vi "GetAncestorClass.vi"(1 "LabVIEWClass":refnum<vi>, 5 "error in (no error)":errorcluster) -> (15 "Ancestor":refnum<vi>, 19 "error out":errorcluster)   [LabVIEW 2017, in "G#IDE.lvlib" / "LibraryLib.lvlib"]
uses:
  LibraryLib.lvlib
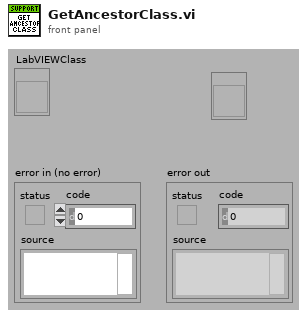
[diagram p1: front panel]
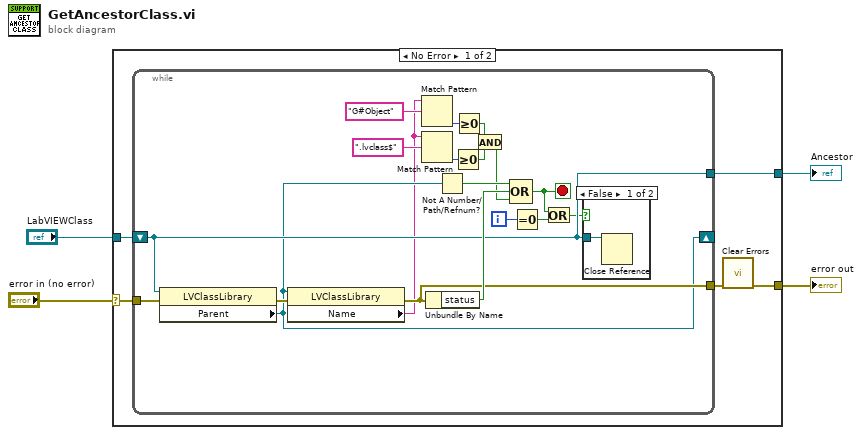
[diagram p0: block diagram]
diagram:
  n1 = case shown="No Error" "error in (no error)" {
    selector: "error in (no error)" -> [w7 w30]
    tunnel: [w6 w30] -> w4
    tunnel: "LabVIEWClass" -> [w9 _]
    tunnel: [w8 _] -> w1
    frame No Error {
      n2 = while {
        shift-right: [w18] -> _
        shift-left: w9 -> [w25]
        tunnel: w7 -> [w26]
        tunnel: [w19] -> w5
        tunnel: [w25] -> w8
        i -> [w22]
        stop <- w24 stop-if-true
        n3 = property class="LVClassLibrary"(reference=w25, error in=w26) -> (error out=w20:errorcluster, "Parent"=w18:refnum<vi>)  [unwired: 1 out]
        n4 = property class="LVClassLibrary"(reference=w18, error in=w20) -> (error out=w19:errorcluster, "Name"=w11:string)  [unwired: 1 out]
        n5 = Match Pattern(string=w11, regular expression="G#Object" ("string")) -> (offset past match=w14:i32)  [unwired: 1 in, 3 out]
        n6 = Match Pattern(string=w11, regular expression=".lvclass$") -> (offset past match=w15:i32)  [unwired: 1 in, 3 out]
        n7 = Unbundle By Name(w19) -> ("status"=w27:bool)
        n8 = Not A Number/Path/Refnum?(number/path/refnum=w18) -> (NaN/Path/Refnum?=w28:bool)
        n9 = Greater Or Equal To 0?(x=w15) -> (x >= 0?=w12:bool)
        n10 = Greater Or Equal To 0?(x=w14) -> (x >= 0?=w13:bool)
        n11 = And(x=w13, y=w12) -> (x .and. y?=w10:bool)
        n12 = Compound Arithmetic op=OR(w28, w27, w10) -> (w24:bool)
        n13 = Equal To 0?(x=w22) -> (x = 0?=w21:bool)
        n14 = Or(x=w24, y=w21) -> (x .or. y?=w23:bool)
        n15 = case shown="False" w23 {
          tunnel: w25 -> [w29 _]
          frame False {
            n16 = Close Reference(reference=w29) -> ()  [unwired: 1 in, 1 out]
          }
          frame True {
          }
        }
      }
      n17 = call <vilib>:"Clear Errors.vi"("error in (no error)"=w5) -> ("error out"=w6:errorcluster)  [unwired: 5 in, 1 out]
    }
    frame Error {
    }
  }
  "error out" <- w4
  "Ancestor" <- w1
